vi "Value Prompt UI.vi"(4 "Max":dbl=inf, 6 "Min":dbl=-inf, 7 "Display Format":string="%.3f", 10 "Default":dbl, 11 "Prompt":string="Enter new value") -> (1 "Cancelled":bool, 2 "New Value":dbl)   [LabVIEW 2020, in "VolatusGUIElements.lvlib" / "DblPopupControl.lvclass"]
uses:
  DblPopupControl.lvclass
  <vilib>/Utility/miscctls.llb/LVSelectionTypeDef.ctl
  DblPopupControl.lvclass/DblPopupControl.ctl
panel:
  in  "Abort Accept":bool
  in  "Cancel":bool
  in  "Accept":bool
  out "Prompt Display":string="Enter new value for\nDuration_s"
  in  "Value":dbl format="%.3f"
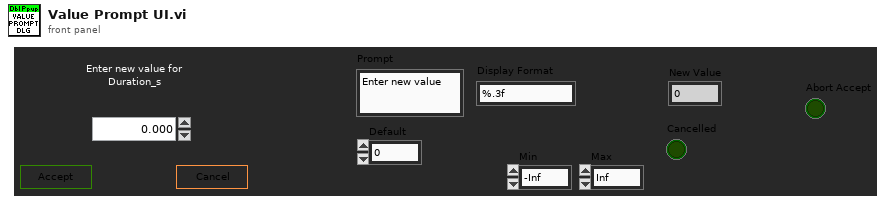
[diagram p1: front panel]
types:
  T1 = typedef "LVSelectionTypeDef.ctl" = cluster{"Selection Start":u32, "Selection End":u32}
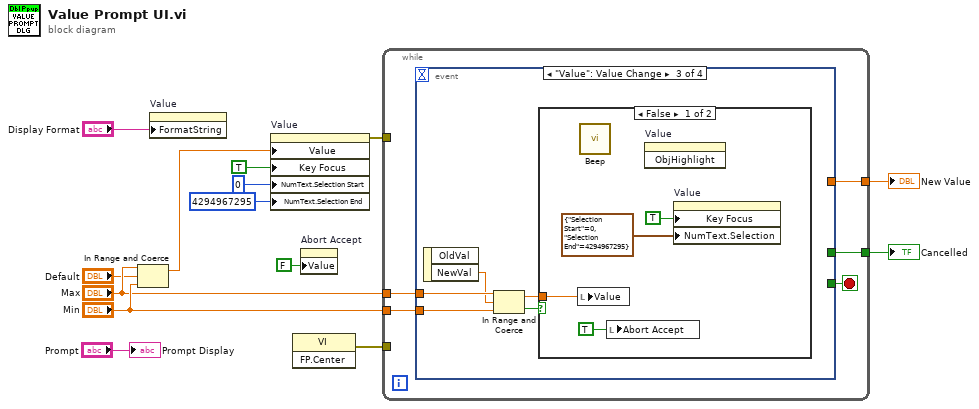
[diagram p0: block diagram]
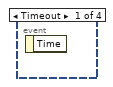
[diagram p2: hidden frame]
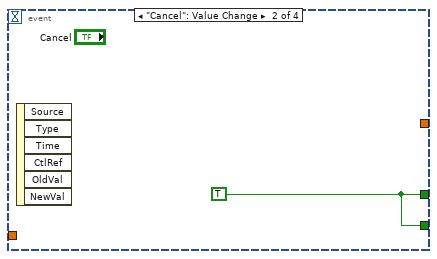
[diagram p3: hidden frame]
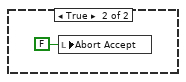
[diagram p4: hidden frame]
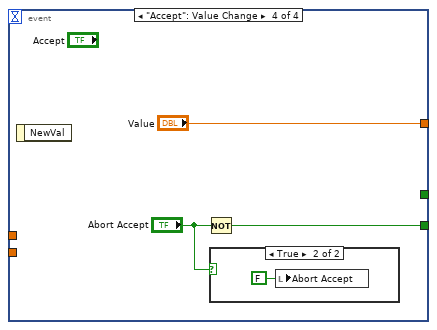
[diagram p5: hidden frame]
diagram:
  n1 = In Range and Coerce(upper limit="Max", x="Default", lower limit="Min") -> (coerced(x)=w2:dbl)  [unwired: 1 out]
  n2 = property on="Value" class="DigNum (strict)"("FormatString"="Display Format") -> ()  [unwired: 2 in, 2 out]
  n3 = property on="Value" class="DigNum (strict)"("Value"=w2, "Key Focus"=TRUE, "NumText.Selection Start"=u32 0 ("Selection Start"), "NumText.Selection End"=u32 4294967295 ("Selection End")) -> (error out=w6:errorcluster)  [unwired: 2 in, 1 out]
  n4 = invoke on="Invoke Node" class="VI" method="FP.Center"() -> (error out=w1:errorcluster)  [unwired: 3 in, 2 out]
  n5 = property on="Abort Accept" class="Bool (strict)"("Value"=FALSE ("Abort Accept")) -> ()  [unwired: 2 in, 2 out]
  n6 = while {
    tunnel: [w19] -> w12
    tunnel: "Max" -> [w17]
    tunnel: "Min" -> [w16]
    tunnel: [w15] -> w7
    tunnel: w6 -> [_]
    tunnel: w1 -> [_]
    stop <- w18 stop-if-true
    n7 = event shown="[2] \"Value\": Value Change" {
      selector: _ -> [_ _ _ _]
      dyn-events: _ -> [_ _ _ _]
      timeout: _ -> [_ _ _ _]
      tunnel: [_ w20 _ _] -> w19
      tunnel: [_ w20 _ w32] -> w18
      tunnel: w17 -> [_ _ w25 _]
      tunnel: w16 -> [_ _ w24 _]
      tunnel: [_ _ _ "Value"] -> w15
      event Timeout {
        n8 = event-data() -> ()  [unwired: 1 in, 1 out]
      }
      event "Cancel": Value Change {
        w20 = TRUE
        n9 = event-data() -> ()  [unwired: 1 in, 6 out]
      }
      event "Value": Value Change {
        n10 = event-data() -> ("NewVal"=w23:dbl)  [unwired: 1 in, 1 out]
        n11 = In Range and Coerce(upper limit=w25, x=w23, lower limit=w24) -> (coerced(x)=w21:dbl, In Range?=w22:bool)
        n12 = case shown="False" w22 {
          tunnel: w21 -> [w29 _]
          frame False {
            n13 = local write "Value"(w29) -> ()
            n14 = call <vilib>:"Beep.vi"() -> ()  [unwired: 12 in]
            n15 = local write "Abort Accept"(TRUE ("Abort Accept")) -> ()
            n16 = invoke on="Value" class="DigNum (strict)" method="ObjHighlight"() -> ()  [unwired: 3 in, 3 out]
            n17 = property on="Value" class="DigNum (strict)"("Key Focus"=TRUE, "NumText.Selection"=T1 {"Selection Start"=0, "Selection End"=4294967295} ("Numeric Text.Selection")) -> ()  [unwired: 2 in, 2 out]
          }
          frame True {
            n18 = local write "Abort Accept"(FALSE ("Abort Accept")) -> ()
          }
        }
      }
      event "Accept": Value Change {
        n19 = event-data() -> ()  [unwired: 1 in, 1 out]
        n20 = Not(x="Abort Accept") -> (.not. x?=w32:bool)
        n21 = case shown="True" "Abort Accept" {
          frame False {
          }
          frame True {
            n22 = local write "Abort Accept"(FALSE ("Abort Accept")) -> ()
          }
        }
      }
    }
  }
  "New Value" <- w7
  "Cancelled" <- w12
  "Prompt Display" <- "Prompt"
